vi "Noise Detector.vi"() -> ()   [LabVIEW 2026]
uses:
  <vilib>/Analysis/baseanly.llb/Mean (DBL).vi
  <vilib>/Analysis/NI_AALBase.lvlib
panel:
  out "Noise Status":string
  out "Average Noise Level":dbl
  out "Signal Comparison":dbl[][](graph)
  in  "Signal Configuration":T1
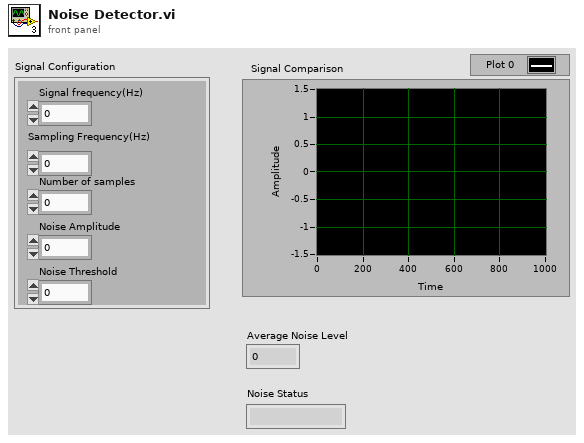
[diagram p1: front panel]
types:
  T1 = cluster{"Signal frequency(Hz)":dbl, "Sampling Frequency(Hz) ":dbl, "Number of samples ":dbl, "Noise Amplitude ":dbl, "Noise Threshold ":dbl}
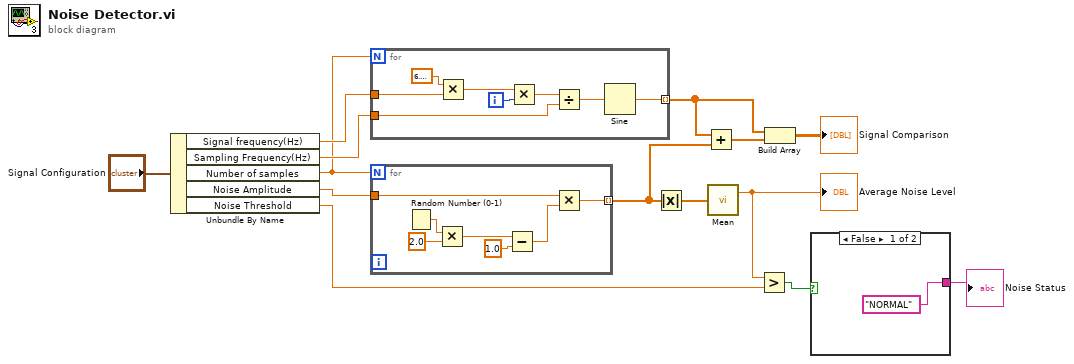
[diagram p0: block diagram]
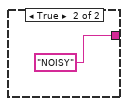
[diagram p2: hidden frame]
diagram:
  n1 = Unbundle By Name("Signal Configuration") -> ("Signal frequency(Hz)"=w13:dbl, "Sampling Frequency(Hz)"=w12:dbl, "Number of samples"=w8:dbl, "Noise Amplitude"=w11:dbl, "Noise Threshold"=w3:dbl)
  n2 = for {
    N: w8 -> [_]
    tunnel: w13 -> [w21]
    tunnel: w12 -> [w17]
    tunnel: [w15] -> w9 mode=indexing
    i -> [w20]
    n3 = Multiply(x=6.283185307179586, y=w21) -> (x*y=w19:dbl)
    n4 = Multiply(x=w19, y=w20) -> (x*y=w18:dbl)
    n5 = Divide(x=w18, y=w17) -> (x/y=w16:dbl)
    n6 = Sine(x=w16) -> (sin(x)=w15:dbl)
  }
  n7 = for {
    N: w8 -> [_]
    tunnel: w11 -> [w24]
    tunnel: [w23] -> w6 mode=indexing
    n8 = Random Number (0-1)() -> (number: 0 to 1=w29:dbl)
    n9 = Multiply(x=w29, y=2.0) -> (x*y=w27:dbl)
    n10 = Subtract(x=w27, y=1.0) -> (x-y=w25:dbl)
    n11 = Multiply(x=w24, y=w25) -> (x*y=w23:dbl)
  }
  n12 = Absolute Value(x=w6) -> (abs(x)=w5:dbl[])
  n13 = Add(x=w9, y=w6) -> (x+y=w10:dbl[])
  n14 = call-poly <vilib>:"Mean.vi"("X"=w5) -> ("mean"=w4:dbl)  [unwired: 1 out]
  "Average Noise Level" <- w4
  n15 = Greater?(x=w4, y=w3) -> (0:w1:bool)
  n16 = Build Array(w9, w10) -> (→"Signal Comparison":dbl[][])
  n17 = case shown="False" w1 {
    tunnel: ["NORMAL" "NOISY"] -> w2
    frame False {
    }
    frame True {
    }
  }
  "Noise Status" <- w2
